vi "RFH-convert-r140.vi"(3 "Xi":dbl[](array[numeric]), 5 "Destination Folder":path, 7 "file path":path, 8 "error in (no error)":errorcluster) -> (0 "error out":errorcluster, 1 "Data":T1, 2 "converted file path":path)   [LabVIEW 2020, in "RFH-Reflection_File_Handler.lvlib"]
doc: "Converts one R140 Excel file to the common format on the frequencies Xi and saves it in the destination folder."
uses:
  RFH-Reflection_File_Handler.lvlib
  RFH-common_data_format.ctl
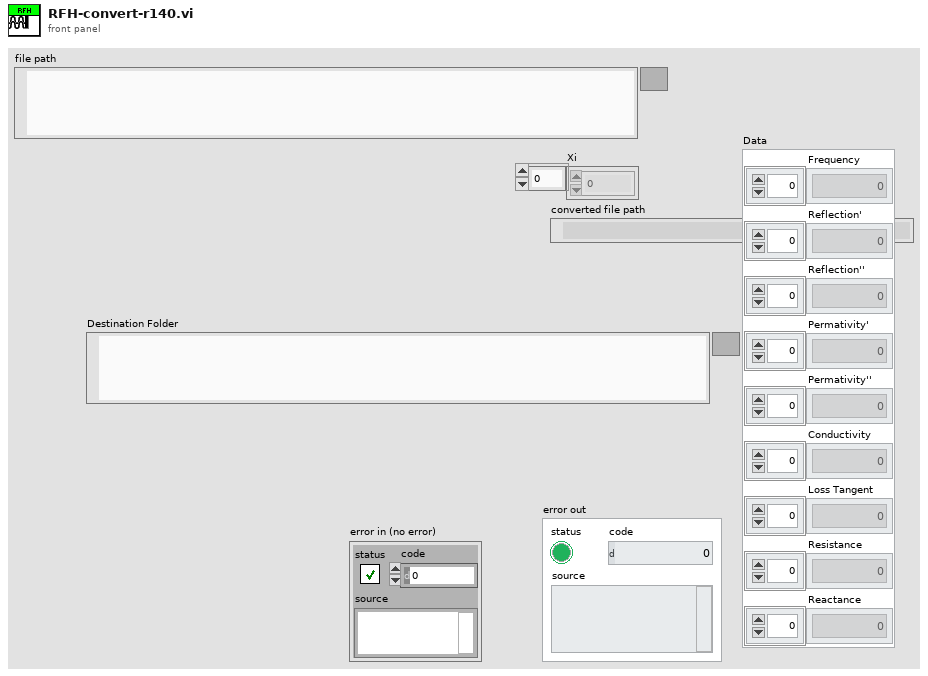
[diagram p1: front panel]
types:
  T1 = typedef "RFH-Reflection_File_Handler.lvlib/RFH-common_data_format.ctl" = cluster{"Frequency":dbl[], "Reflection'":dbl[], "Reflection''":dbl[], "Permativity'":dbl[], "Permativity''":dbl[], "Conductivity":dbl[], "Loss Tangent":dbl[], "Resistance":dbl[], "Reactance":dbl[]}
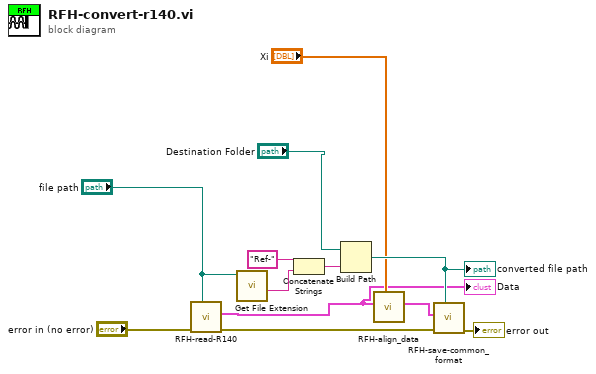
[diagram p0: block diagram]
diagram:
  n1 = call "RFH-read-R140.vi"("file path (dialog if empty)"="file path", "error in (no error)"="error in (no error)") -> ("error out"=w8:errorcluster, "Common Format"=w1:T1)  [unwired: 7 in, 1 out]
  "Data" <- w1
  n2 = call <vilib>:"Get File Extension.vi"("file"="file path") -> ("filename without extension"=w12:string)  [unwired: 6 in, 4 out]
  n3 = Concatenate Strings("Ref-" ("string"), w12) -> (w11:string)
  n4 = Build Path(base path="Destination Folder", name or relative path=w11) -> (appended path=w9:path)
  "converted file path" <- w9
  n5 = call "RFH-align_data.vi"("Xi"="Xi", "Common Format"=w1) -> ("Common Format alligned"=w7:T1)  [unwired: 9 in]
  n6 = call "RFH-save-common_format.vi"("file path (use dialog)"=w9, "error in (no error)"=w8, "Common Format"=w7) -> ("error out"=→"error out":errorcluster)  [unwired: 8 in]
